vi "Update Table.vi"(7 "Limit (10k)":i32=10000 format="%.0p", 8 "error in":errorcluster, 9 "Status Message Ref":refnum<vi>, 10 "New Data in":string[][](array[string]), 11 "Table Data in":string[][](array[string])) -> (0 "error out":errorcluster, 3 "Table Data out":string[][](array[string]))   [LabVIEW 2025, in "Automotive Ethernet Bus Monitor UI.lvlib"]
doc: "Update the table data with new packages. Returns the whole updated data what can be set later."
uses:
  Automotive Ethernet Bus Monitor UI.lvlib
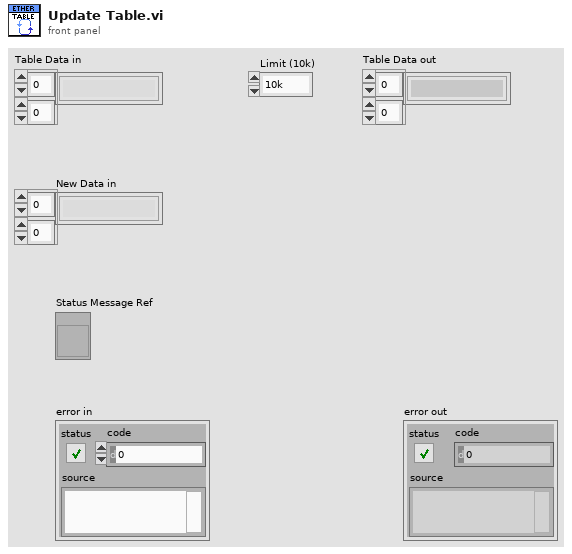
[diagram p1: front panel]
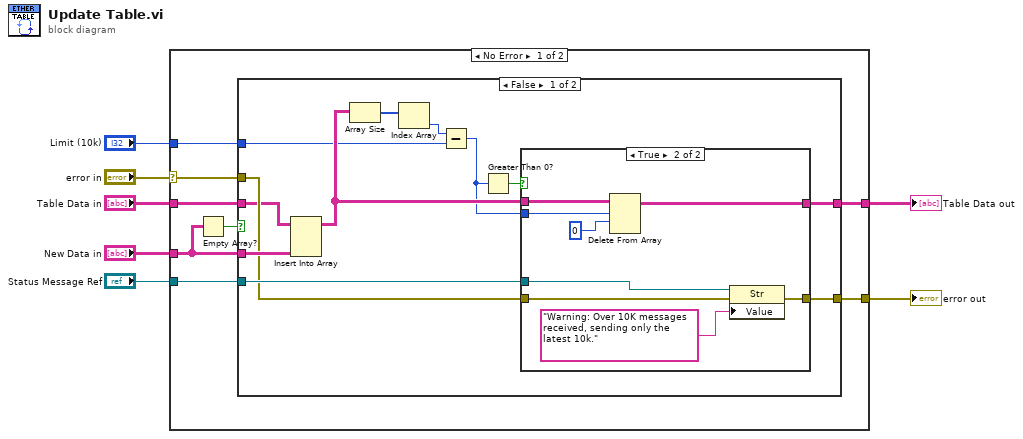
[diagram p0: block diagram]
diagram:
  n1 = case shown="No Error" "error in" {
    selector: "error in" -> [w15 w41]
    tunnel: "New Data in" -> [w12 _]
    tunnel: [w14 w41] -> w5
    tunnel: "Limit (10k)" -> [w11 _]
    tunnel: "Status Message Ref" -> [w10 _]
    tunnel: "Table Data in" -> [w9 w40]
    tunnel: [w8 w40] -> w1
    frame No Error {
      n2 = Empty Array?(array=w12) -> (empty?=w13:bool)
      n3 = case shown="False" w13 {
        tunnel: w12 -> [w27 _]
        tunnel: w15 -> [w19 w39]
        tunnel: [w16 w39] -> w14
        tunnel: w11 -> [w24 _]
        tunnel: w10 -> [w20 _]
        tunnel: w9 -> [w18 w38]
        tunnel: [w17 w38] -> w8
        frame False {
          n4 = Insert Into Array(array=w18, new element=w27) -> (w26:string[][])  [unwired: 2 in]
          n5 = Array Size(array=w26) -> (size(s)=w25:i32[])
          n6 = Index Array(array=w25) -> (element=w21:i32)  [unwired: 1 in]
          n7 = Subtract(x=w21, y=w24) -> (x-y=w22:i32)
          n8 = Greater Than 0?(x=w22) -> (x > 0?=w23:bool)
          n9 = case shown="True" w23 {
            tunnel: w26 -> [w29 w37]
            tunnel: [w29 w36] -> w17
            tunnel: w22 -> [_ w35]
            tunnel: w20 -> [_ w33]
            tunnel: [w28 w31] -> w16
            tunnel: w19 -> [w28 w30]
            frame False {
            }
            frame True {
              n10 = Delete From Array(array=w37, length=w35, index (row)=0) -> (array with subset deleted=w36:string[][])  [unwired: 1 in, 1 out]
              n11 = property on="Property Node" class="Str"(reference=w33, error in=w30, "Value"="Warning: Over 10K messages received, sending only the latest 10k.") -> (error out=w31:errorcluster)  [unwired: 1 out]
            }
          }
        }
        frame True {
        }
      }
    }
    frame Error {
    }
  }
  "error out" <- w5
  "Table Data out" <- w1
